vi "test Error Description from Code.vi"(8 "error in (no error)":errorcluster, 11 "TestCase in":refnum<class "Error Tests.lvclass">) -> (0 "error out":errorcluster, 3 "TestCase out":refnum<class "Error Tests.lvclass">)   [LabVIEW 2020, in "Error Tests.lvclass"]
uses:
  Error Tests.lvclass
  <vilib>/Utility/file.llb/Application Directory.vi
  <vilib>/Utility/libraryn.llb/Check if File or Folder Exists.vi
  <vilib>/addons/_JKI Toolkits/VI Tester/TestCase.llb/TestCase.lvclass
  C:/Program Files/National Instruments/LabVIEW 2024/vi.lib/addons/_JKI Toolkits/VI Tester/TestCase.llb/TestCase.lvclass
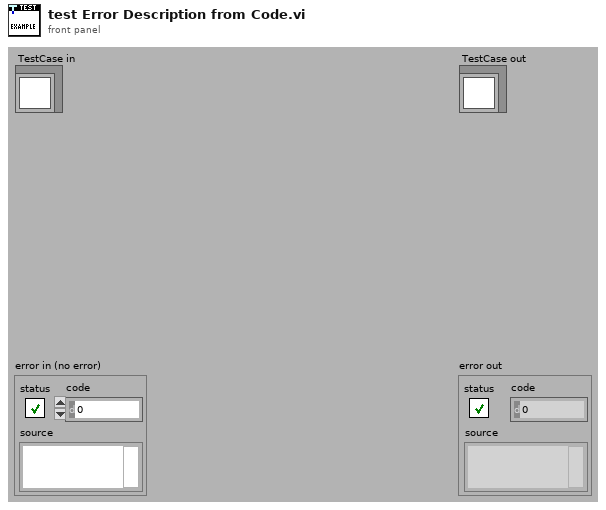
[diagram p1: front panel]
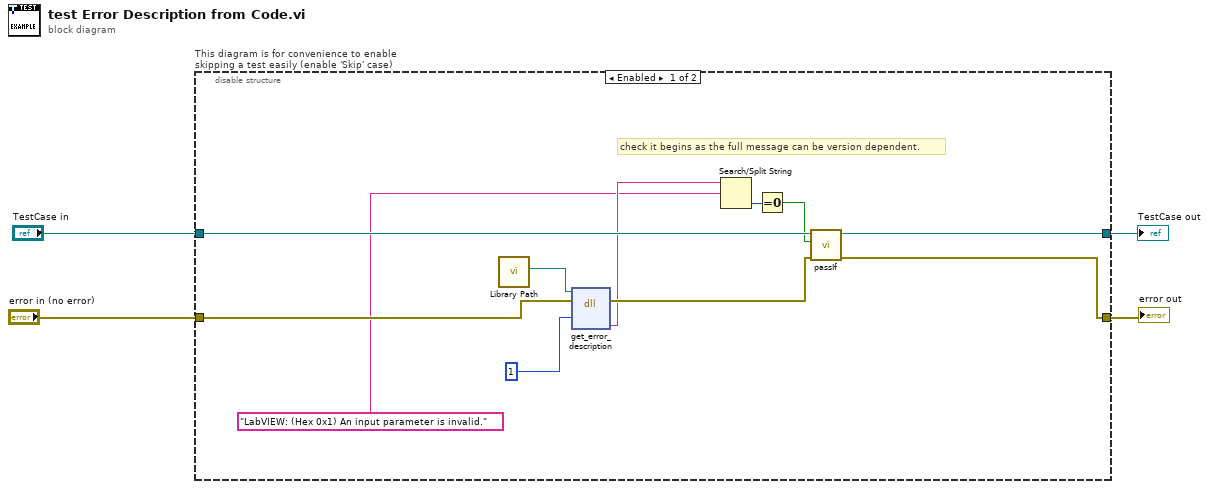
[diagram p0: block diagram]
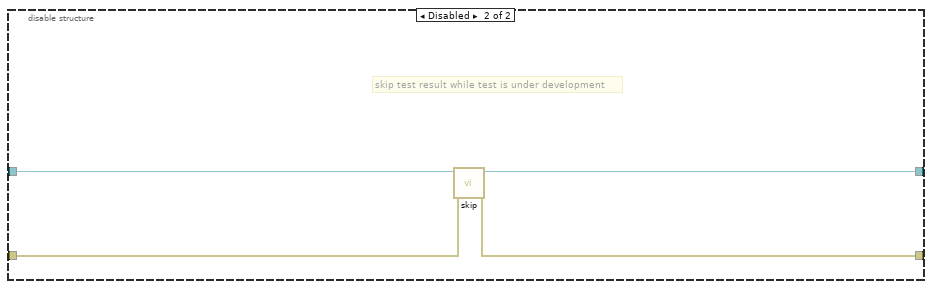
[diagram p2: hidden frame]
diagram:
  n1 = disable-structure "This diagram is for convenience to enable skipping a test easily (enable 'Skip' case)" shown="Enabled" {
    disable-tunnel: "TestCase in" -> [w14 w19]
    disable-tunnel: [w13 w17] -> w1
    disable-tunnel: [w12 w18] -> w3
    disable-tunnel: "error in (no error)" -> [w10 w16]
    frame Enabled {
      # "check it begins as the full message can be version dependent."
      n2 = call "Library Path.vi"() -> ("Library Path"=w15:path)  [unwired: 11 in]
      n3 = dll-call lib="C:/Users/JamesMcNally/Documents/RustInterop/Rust-LabVIEW-Interop/target/debug/labview_test_library.dll" fn="get_error_description"(path in=w15, error in=w10, "code"=1) -> (error out=w11:errorcluster, "description"=w8:string)  [unwired: 4 in, 1 out]
      n4 = Search/Split String(string=w8, search string/char (-)="LabVIEW: (Hex 0x1) An input parameter is invalid.") -> (offset of match=w6:i32)  [unwired: 1 in, 2 out]
      n5 = Equal To 0?(x=w6) -> (x = 0?=w5:bool)
      n6 = call-dynamic "passIf.vi"("error in (no error)"=w11, "pass"=w5, "TestCase in"=w14) -> ("error out"=w12:errorcluster, "TestCase out"=w13:refnum<class "Error Tests.lvclass">)  [unwired: 7 in]
    }
    frame Disabled {
      # "skip test result while test is under development"
      n7 = call <vilib>:"skip.vi"("error in (no error)"=w16, "TestCase in"=w19) -> ("error out"=w18:errorcluster, "TestCase out"=w17:refnum<class "Error Tests.lvclass">)  [unwired: 8 in]
    }
  }
  "error out" <- w3
  "TestCase out" <- w1
